vi "Day 5.vi"() -> ()   [LabVIEW 2021]
uses:
  <vilib>/Utility/file.llb/Read Delimited Spreadsheet (string).vi
  <vilib>/regexp/Match Regular Expression.xnode
panel:
  out "Solution":i32
  out "input":string[](array[string])
  in  "Input File":enum32{"example input", "input"}(radio)
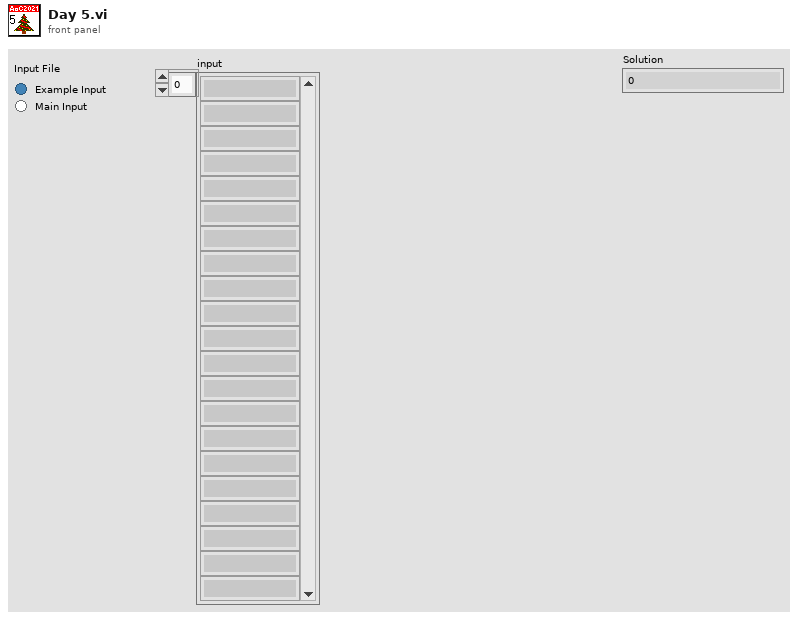
[diagram p1: front panel]
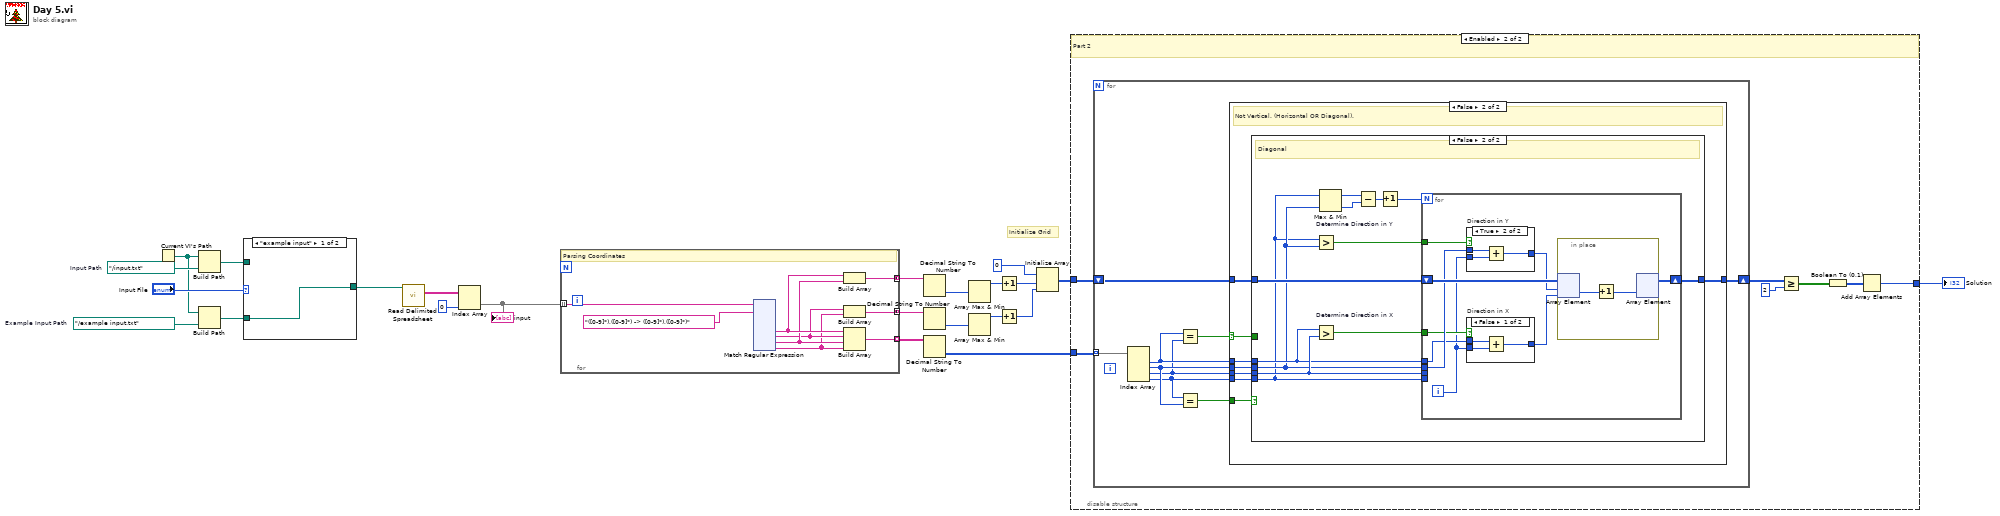
[diagram p0: block diagram]
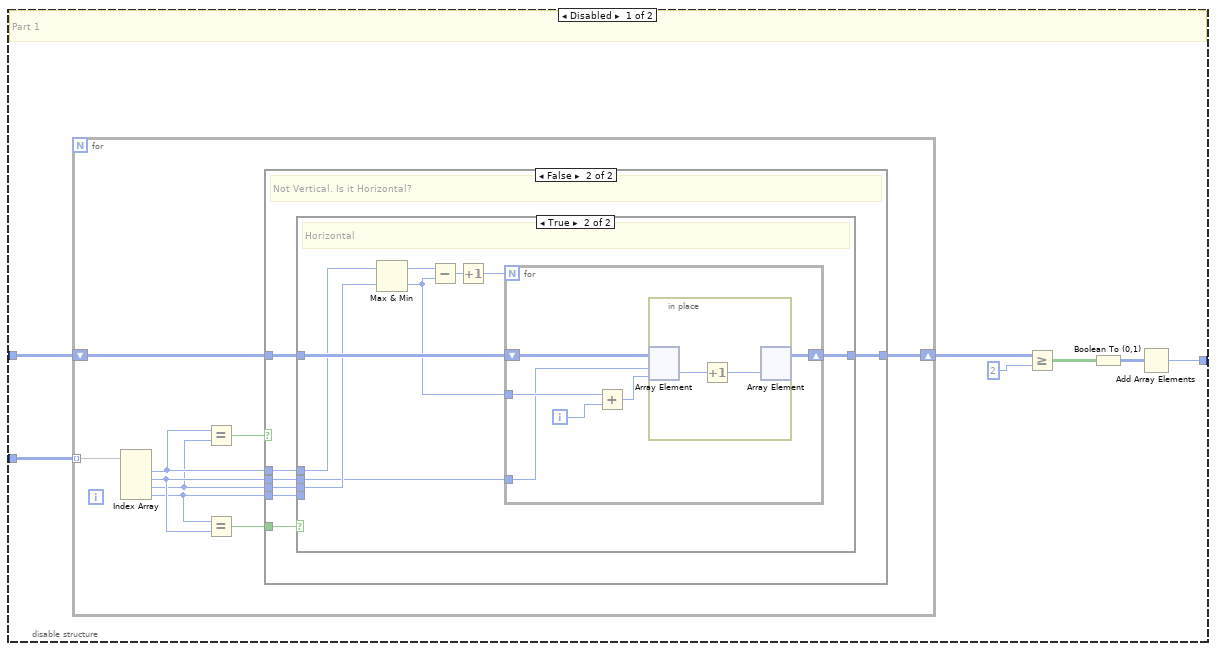
[diagram p3: hidden frame]
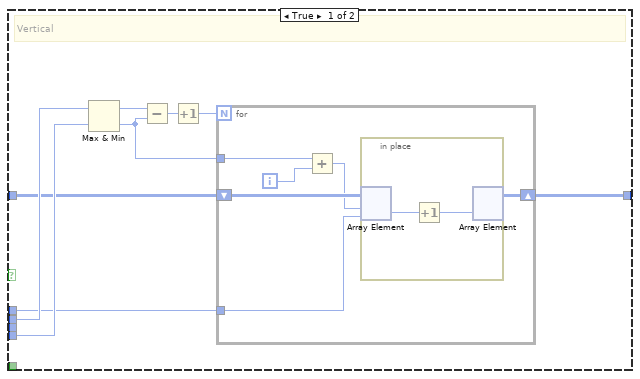
[diagram p4: hidden frame]
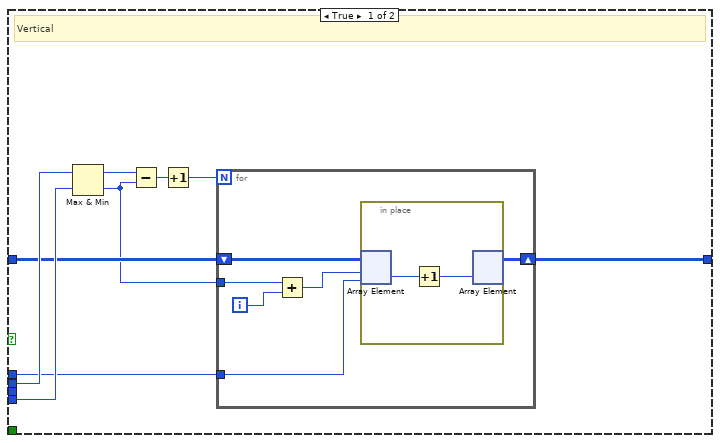
[diagram p6: hidden frame]
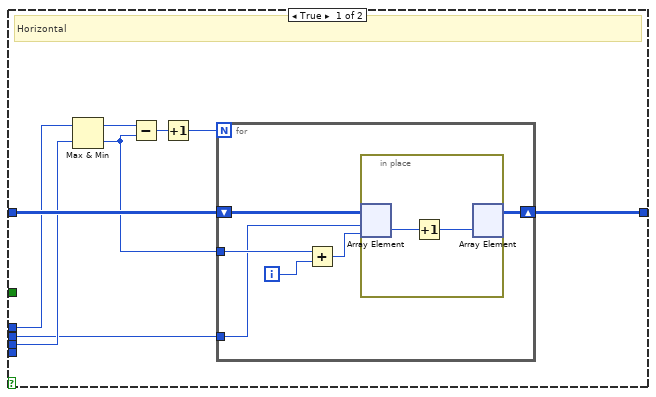
[diagram p7: hidden frame]
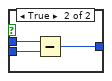
[diagram p8: hidden frame]
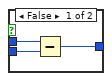
[diagram p9: hidden frame]
diagram:
  w22 = path "../example input.txt"  # Example Input Path
  w23 = path "../input.txt"  # Input Path
  # "Initialize Grid"
  n1 = Current VI's Path() -> (path=w17:path)
  n2 = Build Path(base path=w17, name or relative path=w23) -> (appended path=w20:path)
  n3 = Build Path(base path=w17, name or relative path=w22) -> (appended path=w19:path)
  n4 = case shown="\"example input\"" "Input File" {
    tunnel: w20 -> [_ w25]
    tunnel: w19 -> [w24 _]
    tunnel: [w24 w25] -> w18
    frame "example input" {
    }
    frame "input" {
    }
  }
  n5 = call-poly <vilib>:"Read Delimited Spreadsheet.vi"("file path (dialog if empty)"=w18) -> ("all rows"=w16:string[][])  [unwired: 9 in, 5 out]
  n6 = Index Array(array=w16, index (col)=0 ("disabled index (col)")) -> (element=w14:string[])  [unwired: 1 in]
  "input" <- w14
  n7 = for {
    tunnel: w14 -> [w34] mode=indexing
    tunnel: [w30] -> w13 mode=concatenating
    tunnel: [w29] -> w10 mode=concatenating
    tunnel: [w26] -> w2 mode=indexing
    # "Parsing Coordinates"
    n8 = xnode "Match Regular Expression"("input string"=w34, "regular expression"="([0-9]*),([0-9]*) -> ([0-9]*),([0-9]*)") -> ("submatch 1"=w32:string, "submatch 2"=w28:string, "submatch 3"=w31:string, "submatch 4"=w27:string)  [unwired: 4 in, 5 out]
    n9 = Build Array(w32, w31) -> (w30:string[])
    n10 = Build Array(w28, w27) -> (w29:string[])
    n11 = Build Array(w32, w28, w31, w27) -> (w26:string[])
  }
  n12 = Decimal String To Number(string=w13) -> (number=w12:i32[])  [unwired: 2 in, 1 out]
  n13 = Decimal String To Number(string=w10) -> (number=w11:i32[])  [unwired: 2 in, 1 out]
  n14 = Decimal String To Number(string=w2) -> (number=w1:i32[][])  [unwired: 2 in, 1 out]
  n15 = Array Max & Min(array=w12) -> (max value=w9:i32)  [unwired: 3 out]
  n16 = Array Max & Min(array=w11) -> (max value=w8:i32)  [unwired: 3 out]
  n17 = Increment(x=w9) -> (x+1=w4:i32)
  n18 = Increment(x=w8) -> (x+1=w3:i32)
  n19 = Initialize Array(0, w4, w3) -> (w6:i32[][])
  n20 = disable-structure shown="Enabled" {
    disable-tunnel: w1 -> [w163 w221]
    disable-tunnel: w6 -> [w162 w220]
    disable-tunnel: [w157 w215] -> w5
    frame Disabled {
      # "Part 1"
      n21 = for {
        tunnel: w163 -> [w172] mode=indexing
        shift-right: [w164] -> w161
        shift-left: w162 -> [w167]
        n22 = Index Array(array=w172) -> (element #1=w166:i32, element #2=w170:i32, element #3=w165:i32, element #4=w169:i32)  [unwired: 4 in]
        n23 = Equal?(x=w166, y=w165) -> (x = y?=w171:bool)
        n24 = Equal?(x=w169, y=w170) -> (x = y?=w168:bool)
        n25 = case shown="False" w171 {
          tunnel: w170 -> [w181 w196]
          tunnel: w169 -> [w180 w195]
          tunnel: w168 -> [_ w192]
          tunnel: w167 -> [w177 w194]
          tunnel: w166 -> [w176 w193]
          tunnel: w165 -> [_ w191]
          tunnel: [w174 w190] -> w164
          frame True {
            # "Vertical"
            n26 = Max & Min(x=w181, y=w180) -> (max(x,y)=w179:i32, min(x,y)=w175:i32)
            n27 = Subtract(x=w179, y=w175) -> (x-y=w178:i32)
            n28 = Increment(x=w178) -> (x+1=w173:i32)
            n29 = for {
              N: w173 -> [_]
              shift-right: [w184] -> w174
              shift-left: w177 -> [w187]
              tunnel: w176 -> [w182]
              tunnel: w175 -> [w186]
              i -> [w185]
              n30 = Add(x=w186, y=w185) -> (x+y=w183:i32)
              n31 = in-place {
                n32 = in-place-array #1(w187, w183, w182) -> (w189:i32)
                n33 = Increment(x=w189) -> (x+1=w188:i32)
                n34 = in-place-array #1(w188) -> (w184:i32[][])  [unwired: 2 out]
              }
            }
          }
          frame False {
            # "Not Vertical. Is it Horizontal?"
            n35 = case shown="True" w192 {
              tunnel: w196 -> [_ w200]
              tunnel: w195 -> [_ _]
              tunnel: w194 -> [w197 w204]
              tunnel: w193 -> [_ w202]
              tunnel: w191 -> [_ w201]
              tunnel: [w197 w199] -> w190
              frame False {
              }
              frame True {
                # "Horizontal"
                n36 = Max & Min(x=w202, y=w201) -> (max(x,y)=w206:i32, min(x,y)=w203:i32)
                n37 = Subtract(x=w206, y=w203) -> (x-y=w205:i32)
                n38 = Increment(x=w205) -> (x+1=w198:i32)
                n39 = for {
                  N: w198 -> [_]
                  shift-right: [w209] -> w199
                  shift-left: w204 -> [w212]
                  tunnel: w200 -> [w208]
                  tunnel: w203 -> [w211]
                  i -> [w210]
                  n40 = Add(x=w211, y=w210) -> (x+y=w207:i32)
                  n41 = in-place {
                    n42 = in-place-array #2(w212, w208, w207) -> (w214:i32)
                    n43 = Increment(x=w214) -> (x+1=w213:i32)
                    n44 = in-place-array #2(w213) -> (w209:i32[][])  [unwired: 2 out]
                  }
                }
              }
            }
          }
        }
      }
      n45 = Greater Or Equal?(x=w161, y=2) -> (x >= y?=w159:bool[][])
      n46 = Boolean To (0,1)(Boolean=w159) -> (0, 1=w158:i16[][])
      n47 = Add Array Elements(numeric array=w158) -> (sum=w157:i16)
    }
    frame Enabled {
      # "Part 2"
      n48 = for {
        tunnel: w221 -> [w230] mode=indexing
        shift-right: [w222] -> w219
        shift-left: w220 -> [w225]
        n49 = Index Array(array=w230) -> (element #1=w224:i32, element #2=w228:i32, element #3=w223:i32, element #4=w227:i32)  [unwired: 4 in]
        n50 = Equal?(x=w224, y=w223) -> (x = y?=w229:bool)
        n51 = Equal?(x=w227, y=w228) -> (x = y?=w226:bool)
        n52 = case shown="False" w229 {
          selector: w229 -> [_ w248]
          tunnel: w228 -> [w239 w255]
          tunnel: w227 -> [w238 w254]
          tunnel: w226 -> [_ w251]
          tunnel: w225 -> [w235 w253]
          tunnel: w224 -> [w234 w252]
          tunnel: w223 -> [_ w250]
          tunnel: [w232 w249] -> w222
          frame True {
            # "Vertical"
            n53 = Max & Min(x=w239, y=w238) -> (max(x,y)=w237:i32, min(x,y)=w233:i32)
            n54 = Subtract(x=w237, y=w233) -> (x-y=w236:i32)
            n55 = Increment(x=w236) -> (x+1=w231:i32)
            n56 = for {
              N: w231 -> [_]
              shift-right: [w242] -> w232
              shift-left: w235 -> [w245]
              tunnel: w234 -> [w241]
              tunnel: w233 -> [w244]
              i -> [w243]
              n57 = Add(x=w244, y=w243) -> (x+y=w240:i32)
              n58 = in-place {
                n59 = in-place-array #3(w245, w240, w241) -> (w247:i32)
                n60 = Increment(x=w247) -> (x+1=w246:i32)
                n61 = in-place-array #3(w246) -> (w242:i32[][])  [unwired: 2 out]
              }
            }
          }
          frame False {
            # "Not Vertical. (Horizontal OR Diagonal)."
            n62 = case shown="False" w251 {
              tunnel: w255 -> [w261 w275]
              tunnel: w254 -> [_ w274]
              tunnel: w253 -> [w264 w284]
              tunnel: w252 -> [w263 w280]
              tunnel: w250 -> [w262 w281]
              tunnel: [w260 w283] -> w249
              tunnel: w248 -> [_ _]
              frame True {
                # "Horizontal"
                n63 = Max & Min(x=w263, y=w262) -> (max(x,y)=w259:i32, min(x,y)=w257:i32)
                n64 = Subtract(x=w259, y=w257) -> (x-y=w258:i32)
                n65 = Increment(x=w258) -> (x+1=w256:i32)
                n66 = for {
                  N: w256 -> [_]
                  shift-right: [w267] -> w260
                  shift-left: w264 -> [w270]
                  tunnel: w261 -> [w266]
                  tunnel: w257 -> [w269]
                  i -> [w268]
                  n67 = Add(x=w269, y=w268) -> (x+y=w265:i32)
                  n68 = in-place {
                    n69 = in-place-array #4(w270, w266, w265) -> (w272:i32)
                    n70 = Increment(x=w272) -> (x+1=w271:i32)
                    n71 = in-place-array #4(w271) -> (w267:i32[][])  [unwired: 2 out]
                  }
                }
              }
              frame False {
                # "Diagonal"
                n72 = Greater? "Determine Direction in Y"(x=w274, y=w275) -> (0:w282:bool)
                n73 = Greater? "Determine Direction in X"(x=w280, y=w281) -> (0:w279:bool)
                n74 = Max & Min(x=w274, y=w275) -> (max(x,y)=w278:i32, min(x,y)=w276:i32)
                n75 = Subtract(x=w278, y=w276) -> (x-y=w277:i32)
                n76 = Increment(x=w277) -> (x+1=w273:i32)
                n77 = for {
                  N: w273 -> [_]
                  shift-right: [w292] -> w283
                  shift-left: w284 -> [w293]
                  tunnel: w280 -> [w287]
                  tunnel: w275 -> [w290]
                  tunnel: w281 -> [_]
                  tunnel: w282 -> [w289]
                  tunnel: w274 -> [_]
                  tunnel: w279 -> [w288]
                  i -> [w286]
                  n78 = case "Direction in Y" shown="True" w289 {
                    tunnel: w286 -> [w301 w305]
                    tunnel: [w300 w304] -> w291
                    tunnel: w290 -> [w302 w303]
                    frame False {
                      n79 = Subtract(x=w302, y=w301) -> (x-y=w300:i32)
                    }
                    frame True {
                      n80 = Add(x=w303, y=w305) -> (x+y=w304:i32)
                    }
                  }
                  n81 = case "Direction in X" shown="False" w288 {
                    tunnel: w286 -> [w296 w298]
                    tunnel: [w295 w297] -> w285
                    tunnel: w287 -> [w294 w299]
                    frame False {
                      n82 = Add(x=w294, y=w296) -> (x+y=w295:i32)
                    }
                    frame True {
                      n83 = Subtract(x=w299, y=w298) -> (x-y=w297:i32)
                    }
                  }
                  n84 = in-place {
                    n85 = in-place-array #5(w293, w291, w285) -> (w307:i32)
                    n86 = Increment(x=w307) -> (x+1=w306:i32)
                    n87 = in-place-array #5(w306) -> (w292:i32[][])  [unwired: 2 out]
                  }
                }
              }
            }
          }
        }
      }
      n88 = Greater Or Equal?(x=w219, y=2) -> (x >= y?=w217:bool[][])
      n89 = Boolean To (0,1)(Boolean=w217) -> (0, 1=w216:i16[][])
      n90 = Add Array Elements(numeric array=w216) -> (sum=w215:i16)
    }
  }
  "Solution" <- w5
